vi "DriverStation Get Mode And Status.vi"(11 "Occurrence Refnum":refnum<k4>) -> (0 "OutputsEnabled?":bool, 1 "RobotMode":u8, 2 "Match Time(s)":sgl, 3 "currentOpMode":u64, 4 "details":T1, 5 "Enabled":bool)   [LabVIEW 2023, in "MrcLib.lvlib"]
doc: "This VI returns the operating mode and status of the robot. If an occurrence is passed in, it delays until the DS sends the next packet."
uses:
  <vilib>/MRC/MrcLib.lvlib
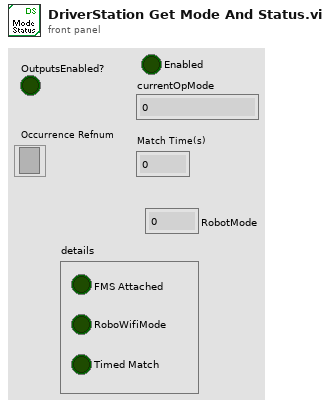
[diagram p1: front panel]
types:
  T1 = cluster{"FMS Attached":bool, "RoboWifiMode":bool, "Timed Match":bool}
  T2 = typedef "MrcLib.lvlib/MRC_ControlData.ctl" = cluster{"controlFlags":u32, "matchTime":u16, "currentOpMode":u64, "gameDataLength":u8, "game data":T3}
  T3 = typedef "MRC Str64.ctl" = cluster{"[0]":u8, "[1]":u8, "[2]":u8, "[3]":u8, "[4]":u8, "[5]":u8, "[6]":u8, "[7]":u8, "[8]":u8, "[9]":u8, "[10]":u8, "[11]":u8, "[12]":u8, "[13]":u8, "[14]":u8, "[15]":u8, "[16]":u8, "[17]":u8, "[18]":u8, "[19]":u8, "[20]":u8, "[21]":u8, "[22]":u8, "[23]":u8, "[24]":u8, "[25]":u8, "[26]":u8, "[27]":u8, "[28]":u8, "[29]":u8, "[30]":u8, "[31]":u8, "[32]":u8, "[33]":u8, "[34]":u8, "[35]":u8, "[36]":u8, "[37]":u8, "[38]":u8, "[39]":u8, "[40]":u8, "[41]":u8, "[42]":u8, "[43]":u8, "[44]":u8, "[45]":u8, "[46]":u8, "[47]":u8, "[48]":u8, "[49]":u8, "[50]":u8, "[51]":u8, "[52]":u8, "[53]":u8, "[54]":u8, "[55]":u8, "[56]":u8, "[57]":u8, "[58]":u8, "[59]":u8, "[60]":u8, "[61]":u8, "[62]":u8, "[63]":u8}
  T4 = cluster{"FMSConnected":bool, "SupportOpModes":bool, "Alliance":u32, "RoboWifiMode":bool, "Timed Match":bool, "DS Connected":bool}
  T5 = cluster{"FMSConnected":bool, "RoboWifiMode":bool, "Timed Match":bool}
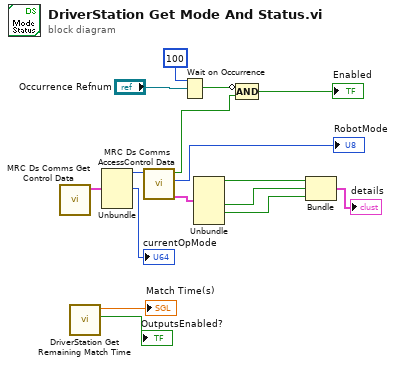
[diagram p0: block diagram]
diagram:
  n1 = call <vilib>:"MRC Ds Comms Get Control Data.vi"() -> ("data out"=w15:T2)  [unwired: 10 in, 1 out]
  n2 = call <vilib>:"DriverStation Get Remaining Match Time.vi"() -> ("OutputsEnabled?"=→"OutputsEnabled?":bool, "Match Time(s)"=→"Match Time(s)":sgl)  [unwired: 9 in, 1 out]
  n3 = Unbundle(w15) -> ("controlFlags"=w14:u32, "currentOpMode"=→"currentOpMode":u64)  [unwired: 3 out]
  n4 = call <vilib>:"MRC Ds Comms AccessControl Data.vi"("controlFlag"=w14) -> ("info"=w16:T4, "RobotMode"=→"RobotMode":u8, "Enabled"=w2:bool)  [unwired: 7 in, 1 out]
  n5 = Wait on Occurrence(2:"Occurrence Refnum", 3:100 ("ms timeout (-1)")) -> (0:w3:bool)  [unwired: 1 in]
  n6 = Unbundle(w16) -> ("FMSConnected"=w12:bool, "RoboWifiMode"=w11:bool, "Timed Match"=w10:bool)  [unwired: 3 out]
  n7 = Compound Arithmetic op=AND(invert w3, w2) -> (→"Enabled":bool)
  n8 = Bundle("FMSConnected"=w12, "RoboWifiMode"=w11, "Timed Match"=w10) -> (→"details":T5)  [unwired: 1 in]
